vi "Highscore_Insert.vi"(0 "Table":cluster{"Score":i32, "Name":string}[](array[cluster]), 5 "Score":i32, 7 "Name":string, 11 "error in":errorcluster) -> (4 "Table out":cluster{"Score":i32, "Name":string}[](array[cluster]), 15 "error out":errorcluster)   [LabVIEW 2020, in "GH_Engine.lvlib"]
doc: "Inserts Score and Name into the list, sorts it (best first) and keeps the best 5."
uses:
  GH_Engine.lvlib
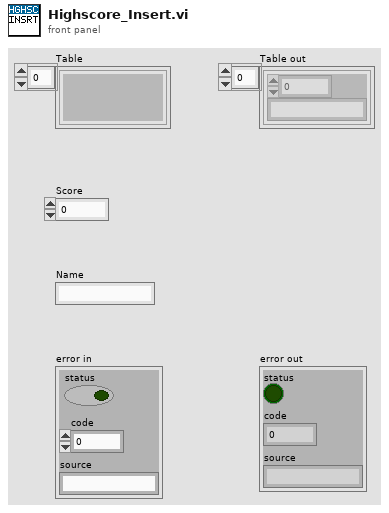
[diagram p1: front panel]
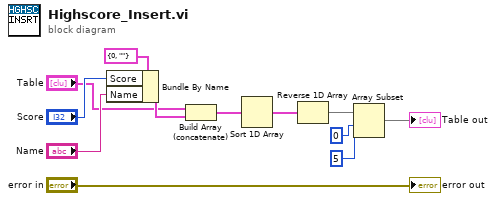
[diagram p0: block diagram]
diagram:
  n1 = Bundle By Name(cluster=cluster{"Score":i32, "Name":string} {"Score"=0, "Name"=""}, "Score"="Score", "Name"="Name") -> (w6:cluster{"Score":i32, "Name":string})
  n2 = Build Array (concatenate)("Table", w6) -> (w7:cluster{"Score":i32, "Name":string}[])
  n3 = Sort 1D Array(array=w7) -> (sorted array=w8:cluster{"Score":i32, "Name":string}[])
  n4 = Reverse 1D Array(array=w8) -> (reversed array=w9:cluster{"Score":i32, "Name":string}[])
  n5 = Array Subset(array=w9, index=0, length=5) -> (→"Table out":cluster{"Score":i32, "Name":string}[])
  "error out" <- "error in"
